vi "KYFG Buffer Get Size.vi"(8 "error in (no error)":errorcluster, 11 "buffHandle":u32) -> (0 "error out":errorcluster, 2 "buffer size":u64, 3 "buffHandle out":u32)   [LabVIEW 2023, in "KYFGLib_lv.lvlib"]
doc: "KYFG_API long long KYFG_BufferGetSize(BUFFHANDLE buffHandle);"
uses:
  KYFGLib_lv.lvlib
  KYFGLib.dll
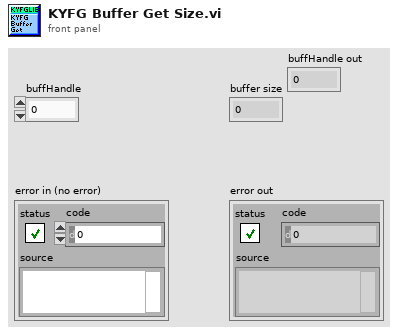
[diagram p1: front panel]
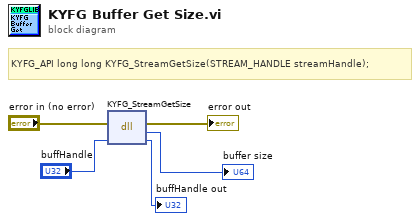
[diagram p0: block diagram]
diagram:
  # "KYFG_API long long\tKYFG_StreamGetSize(STREAM_HANDLE streamHandle);"
  n1 = dll-call lib="KYFGLib.dll" fn="KYFG_StreamGetSize"(error in="error in (no error)", "streamHandle"="buffHandle") -> (error out=→"error out":errorcluster, "return type"=→"buffer size":u64, "streamHandle"=→"buffHandle out":u32)  [unwired: 2 in, 1 out]
